vi "Add Relay Channel.vi"(8 "error in (no error)":errorcluster, 10 "Relay Channel Data":T2, 11 "MUX Section Ref in":T1 format="%.0x") -> (0 "error out":errorcluster, 3 "MUX Section Ref out":T1 format="%.0x")   [LabVIEW 2013, in "MUX Custom Device.lvlib"]
uses:
  MUX Custom Device.lvlib
  <vilib>/NI Veristand/Custom Device API/Custom Device Item Ref.ctl
  Relay Channel Data.ctl
  Relay Data.ctl
  Switch.ctl
  <vilib>/NI Veristand/Custom Device API/Custom Device Channel.ctl
  <vilib>/NI Veristand/Custom Device API/Custom Device Channel Type.ctl
  MUX Global.vi
  <vilib>/NI Veristand/Custom Device API/Set Item Property (String).vi
  <vilib>/NI Veristand/Custom Device API/Custom Device API.lvlib
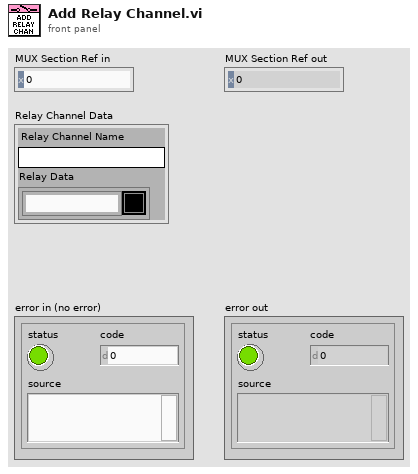
[diagram p1: front panel]
types:
  T1 = typedef "Custom Device API.lvlib/Custom Device Item Ref.ctl" = u64
  T2 = typedef "MUX Custom Device.lvlib/Relay Channel Data.ctl" = cluster{"Relay Channel Name":string, "Relay Data":T3}
  T3 = typedef "MUX Custom Device.lvlib/Relay Data.ctl" = cluster{"Relay Name":string, "State":T4}
  T4 = typedef "MUX Custom Device.lvlib/Switch.ctl" = bool
  T5 = typedef "Custom Device API.lvlib/Custom Device Channel.ctl" = cluster{"Type":T6, "Units":string, "Default Value":dbl, "Faultable":bool, "Scalable":bool}
  T6 = typedef "Custom Device API.lvlib/Custom Device Channel Type.ctl" = enum16{"Input", "Output"}
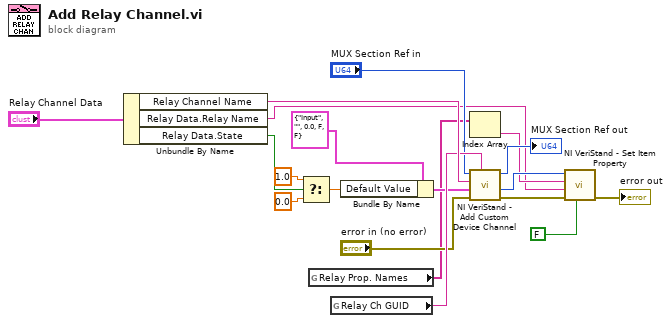
[diagram p0: block diagram]
diagram:
  n1 = Unbundle By Name("Relay Channel Data") -> ("Relay Channel Name"=w19:string, "Relay Data.Relay Name"=w2:string, "Relay Data.State"=w12:T4)
  n2 = Select(t=1.0, s=w12, f=0.0) -> (s? t:f=w16:dbl)
  n3 = global read "MUX Global.vi" "Relay Prop. Names"() -> (w4:string[])
  n4 = global read "MUX Global.vi" "Relay Ch GUID"() -> (w18:string)
  n5 = Bundle By Name(cluster=T5 {"Type"=enum."Input", "Units"="", "Default Value"=0.0, "Faultable"=FALSE, "Scalable"=FALSE} ("Channel"), "Default Value"=w16) -> (w17:T5)
  n6 = Index Array(array=w4) -> (element=w3:string)  [unwired: 1 in]
  n7 = call <vilib>:"NI VeriStand - Add Custom Device Channel.vi"("GUID (Default Channel)"=w18, "error in (no error)"="error in (no error)", "Channel"=w17, "Channel Name"=w19, "Parent Ref in"="MUX Section Ref in") -> ("error out"=w7:errorcluster, "Channel Ref"=w6:T1, "Parent Ref out"=→"MUX Section Ref out":T1)  [unwired: 3 in, 1 out]
  n8 = call-poly <vilib>:"NI VeriStand - Set Item Property.vi"("Binary String (T)"=FALSE, "error in (no error)"=w7, "Value"=w2, "Property Name"=w3, "Item Ref in"=w6) -> ("error out"=→"error out":errorcluster)  [unwired: 4 in, 2 out]
